vi "control Remote Connection Error.vi"(8 "error in (no error)":errorcluster, 11 "FSV-40N in":refnum<class "FSV-40N.lvclass">) -> (0 "error out":errorcluster, 3 "FSV-40N out":refnum<class "FSV-40N.lvclass">)   [LabVIEW 2023, in "Spectrum Analyzer.lvlib" / "FSV-40N.lvclass"]
uses:
  FSV-40N.lvclass
  FSV-40N.lvclass/FSV-40N.ctl
  <vilib>/ErrorRing/Error Ring.xnode
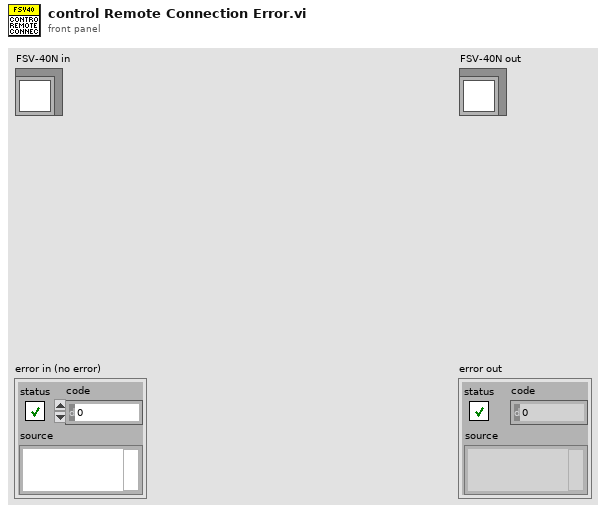
[diagram p1: front panel]
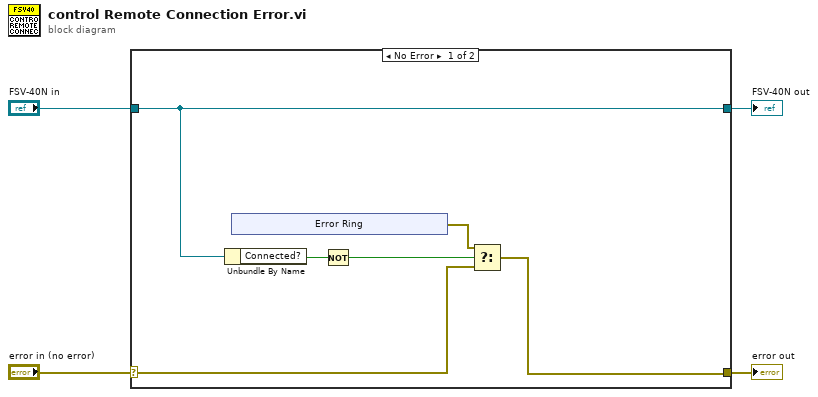
[diagram p0: block diagram]
diagram:
  n1 = case shown="No Error" "error in (no error)" {
    selector: "error in (no error)" -> [w6 w13]
    tunnel: [w5 w13] -> w3
    tunnel: [w10 w12] -> w1
    tunnel: "FSV-40N in" -> [w10 w12]
    frame No Error {
      n2 = Unbundle By Name(w10) -> ("Connected?"=w9:bool)
      n3 = xnode "Error Ring"() -> ("error out"=w7:errorcluster)
      n4 = Not(x=w9) -> (.not. x?=w8:bool)
      n5 = Select(t=w7, s=w8, f=w6) -> (s? t:f=w5:errorcluster)
    }
    frame Error {
    }
  }
  "error out" <- w3
  "FSV-40N out" <- w1
